vi "Fix Duplicates in Tree.vi"(8 "error in (no error)":errorcluster, 11 "Data in":T1={"PeekVI Reference"=refnum, "SubPanel"=refnum, "Peek Stack Tree Ref"=refnum, "Open Button Ref"=refnum, "Top VI"=refnum, "Active VI"=refnum, "Stack"=[], "Last FP State"=enum."Standard"}) -> (0 "error out":errorcluster, 3 "Data out":T1={"PeekVI Reference"=refnum, "SubPanel"=refnum, "Peek Stack Tree Ref"=refnum, "Open Button Ref"=refnum, "Top VI"=refnum, "Active VI"=refnum, "Stack"=[], "Last FP State"=enum."Standard"})   [LabVIEW 2020, in "Peek Window.lvlib"]
uses:
  Peek Window.lvlib
  MHL Data Cluster.ctl
  VI Types/Standard VI Type/Standard VI Type.lvclass
  VI Types/Standard VI Type/Standard VI Type.lvclass/Standard VI Type.ctl
  VI Types/Standard VI Type/Read Full Qualified Name.vi
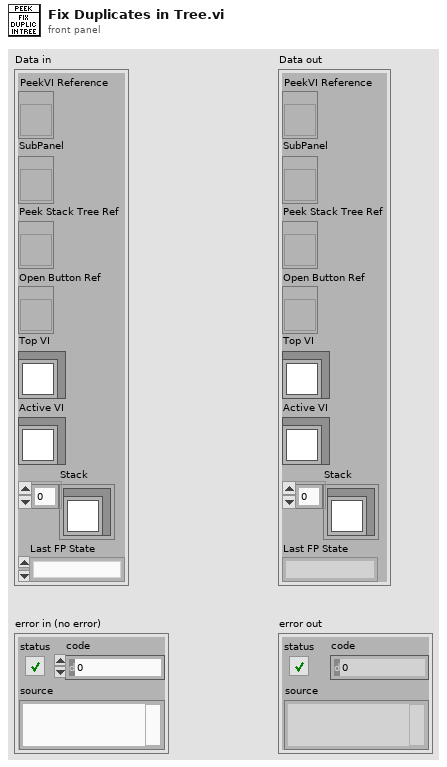
[diagram p1: front panel]
types:
  T1 = typedef "Peek Window.lvlib/MHL Data Cluster.ctl" = cluster{"PeekVI Reference":refnum<vi>, "SubPanel":refnum<vi>, "Peek Stack Tree Ref":refnum<vi>, "Open Button Ref":refnum<vi>, "Top VI":refnum<class "Standard VI Type.lvclass">, "Active VI":refnum<class "Standard VI Type.lvclass">, "Stack":refnum<class "Standard VI Type.lvclass">[], "Last FP State":enum32{"Invalid", "Standard", "Closed", "Hidden", "Minimized", "Maximized"}}
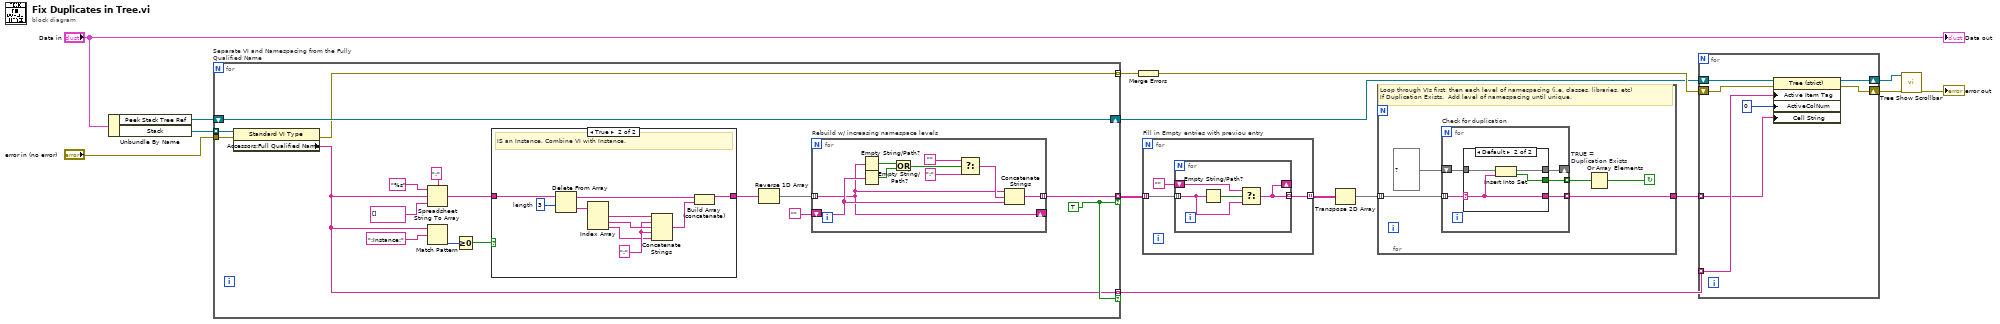
[diagram p0: block diagram]
diagram:
  n1 = Unbundle By Name("Data in") -> ("Peek Stack Tree Ref"=w9:refnum<vi>, "Stack"=w10:refnum<class "Standard VI Type.lvclass">[])
  n2 = for "Separate VI and Namespacing from the Fully Qualified Name" {
    tunnel: [w32] -> w6 mode=indexing if=w29
    tunnel: w10 -> [w30] mode=indexing
    tunnel: [w21] -> w11 mode=indexing if=w29
    tunnel: [w22] -> w8 mode=indexing
    tunnel: "error in (no error)" -> [w23]
    shift-right: [w31] -> w4
    shift-left: w9 -> [w31]
    w29 = TRUE
    n3 = property class="Standard VI Type"(reference=w30, error in=w23) -> (error out=w22:errorcluster, "Accessors:Full Qualified Name"=w21:string)  [unwired: 1 out]
    n4 = Spreadsheet String To Array(delimiter (Tab)=":", format string="%s", spreadsheet string=w21, array type (2D Dbl)=string[] []) -> (array=w25:string[])
    n5 = Match Pattern(string=w21, regular expression=":Instance:") -> (offset past match=w19:i32)  [unwired: 1 in, 3 out]
    n6 = Greater Or Equal To 0?(x=w19) -> (x >= 0?=w18:bool)
    n7 = case shown="True" w18 {
      tunnel: w25 -> [w33 w43]
      tunnel: [w33 w35] -> w17
      frame False {
        # "NOT an Instance"
      }
      frame True {
        w38 = ":"
        w42 = 3  # length
        # "IS an Instance. Combine VI with Instance."
        n8 = Delete From Array(array=w43, length=w42) -> (deleted portion=w41:string[], array with subset deleted=w36:string[])  [unwired: 1 in]
        n9 = Index Array(array=w41) -> (element #1=w40:string, element #2=w39:string, element #3=w37:string)  [unwired: 3 in]
        n10 = Concatenate Strings(w40, w38, w39, w38, w37) -> (w34:string)
        n11 = Build Array (concatenate)(w36, w34) -> (w35:string[])
      }
    }
    n12 = Reverse 1D Array(array=w17) -> (reversed array=w16:string[])
    n13 = for "Rebuild w/ increasing namespace levels" {
      tunnel: w16 -> [w47] mode=indexing
      shift-right: [w47] -> _
      shift-left: "" -> [w51]
      tunnel: [w52] -> w32 mode=indexing
      n14 = Empty String/Path?(string/path=w47) -> (empty?=w46:bool)
      n15 = Empty String/Path?(string/path=w51) -> (empty?=w45:bool)
      n16 = Or(x=w46, y=w45) -> (x .or. y?=w44:bool)
      n17 = Select(t="", s=w44, f=":") -> (s? t:f=w48:string)
      n18 = Concatenate Strings(w47, w48, w51) -> (w52:string)
    }
  }
  n19 = Merge Errors(w8) -> (w13:errorcluster)
  n20 = for "Fill in Empty entries with previou entry" {
    tunnel: w6 -> [w55] mode=indexing
    tunnel: [w54] -> w7 mode=indexing
    n21 = for {
      tunnel: w55 -> [w58] mode=indexing
      tunnel: [w57] -> w54 mode=indexing
      shift-right: [w57] -> _
      shift-left: "" -> [w56]
      n22 = Empty String/Path?(string/path=w58) -> (empty?=w59:bool)
      n23 = Select(t=w56, s=w59, f=w58) -> (s? t:f=w57:string)
    }
  }
  n24 = Transpose 2D Array(2D array=w7) -> (transposed array=w5:string[][])
  n25 = for {
    tunnel: w5 -> [w64] mode=indexing
    tunnel: [w60] -> w12
    stop <- w61 continue-if-true
    # "Loop through VIs first, then each level of namespacing (i.e. classes, libraries, etc)\nIf Duplication Exists.  Add level of namespacing until unique."
    n26 = for "Check for duplication" {
      tunnel: w64 -> [w68] mode=indexing
      shift-right: [w66] -> _
      shift-left: set{string} {} ("set in") -> [w69]
      tunnel: [w67] -> w62 mode=indexing
      tunnel: [w65] -> w60 mode=indexing
      n27 = case shown="Default" w68 {
        selector: w68 -> [w70 w72]
        tunnel: w69 -> [w71 w74]
        tunnel: [_ w75] -> w67
        tunnel: [w71 w73] -> w66
        tunnel: [w70 w72] -> w65
        frame "" {
        }
        frame Default {
          n28 = Insert Into Set(10:w72, 11:w74) -> (2:w75:bool, 3:w73:set{string})
        }
      }
    }
    n29 = Or Array Elements "TRUE =\nDuplication Exists"(Boolean array=w62) -> (logical OR=w61:bool)
  }
  n30 = for {
    shift-right: [w80] -> w1
    shift-left: w4 -> [w82]
    tunnel: w11 -> [w79] mode=indexing
    tunnel: w12 -> [w77] mode=indexing
    shift-right: [w76] -> w3
    shift-left: w13 -> [w81]
    n31 = property class="Tree (strict)"(reference=w82, error in=w81, "Active Item Tag"=w79, "ActiveColNum"=0, "Cell String"=w77) -> (reference out=w80:refnum<vi>, error out=w76:errorcluster)
  }
  n32 = call "Tree Show Scrollbar.vi"("error in (no error)"=w3, "Tree"=w1) -> ("error out"=→"error out":errorcluster)  [unwired: 8 in, 1 out]
  "Data out" <- "Data in"
